vi "to string array.vi"(8 "error in (no error)":errorcluster, 11 "module configuration in":refnum<class "Daqmx Module configuration.lvclass">) -> (0 "error out":errorcluster, 1 "Array":string[][](array[string]), 2 "version":string, 3 "module configuration out":refnum<class "Daqmx Module configuration.lvclass">)   [LabVIEW 2015, in "DAQmx Module Configuration.lvclass"]
uses:
  Daqmx Module configuration.lvclass
  Daqmx Module configuration.lvclass/Daqmx Module configuration.ctl
  <vilib>/NI/Tag Bus/tag/tag descriptor.lvclass/tag descriptor.ctl
  <vilib>/NI/Tag Bus Module Framework/module configuration/TBM module configuration.lvclass
  <vilib>/NI/Tag Bus/tag/tag descriptor.lvclass
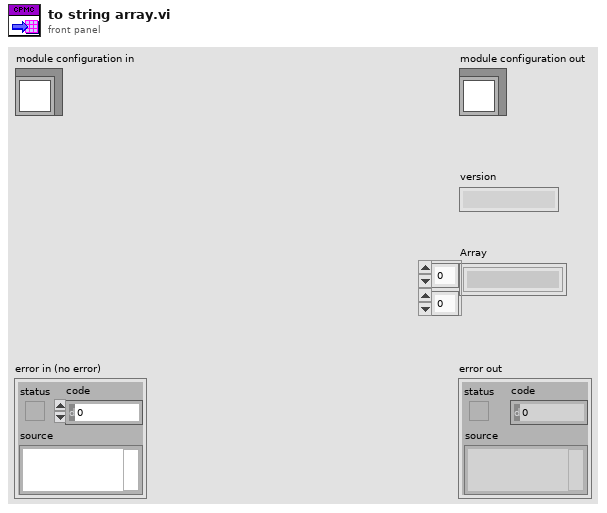
[diagram p1: front panel]
types:
  T1 = typedef "DAQmx Module Configuration.lvclass/Line.ctl" = cluster{"Channel Array":refnum<class "TBM channel.lvclass">[], "Physical Channel":string, "Measurement Type":T2, "Parameters":T3}
  T2 = typedef "DAQmx Module Configuration.lvclass/Measurement Type.ctl" = enum16{"Digital Input", "Digital Output", "Voltage Input", "Voltage Output", "Current Input", "Current Output", "RTD", "Thermocouple", "Strain", "PWM"}
  T3 = typedef "DAQmx Module Configuration.lvclass/Parameters.ctl" = cluster{"Digital Config":cluster{"Invert Lines?":bool}, "Voltage Config":cluster{"Maximum Value (V)":dbl, "Minimum Value (V)":dbl, "in terminal configuration (V)":i32, "out terminal configuration (V)":i32}, "Current Config":cluster{"Maximum Value (A)":dbl, "Minimum Value (A)":dbl, "shunt resistor location":i32, "input terminal configuration (C)":i32, "external shunt resistor value":dbl}, "RTD Config":cluster{"Maximum Value (°C)":dbl, "Minimum Value (°C)":dbl, "resistance configuration":i32, "r0":dbl, "current excitation value":dbl, "rtd type":i32, "current excitation source":i32}, "Thermocouple Config":cluster{"Minimum Value (C)":dbl, "Maximum Value (C)":dbl, "thermocouple type":i32, "cjc source":i32, "cjc value":dbl}, "Strain Config":cluster{"Maximum Value":dbl, "Minimum Value":dbl, "bridge information":cluster{"strain configuration":i32, "lead wire resistance":dbl, "initial bridge voltage":dbl, "voltage excitation source":i32, "voltage excitation value":dbl}, "strain gage information":cluster{"gage factor":dbl, "nominal gage resistance":dbl, "poisson ratio":dbl}}, "PWM Config":cluster{"Idle State":bool}}
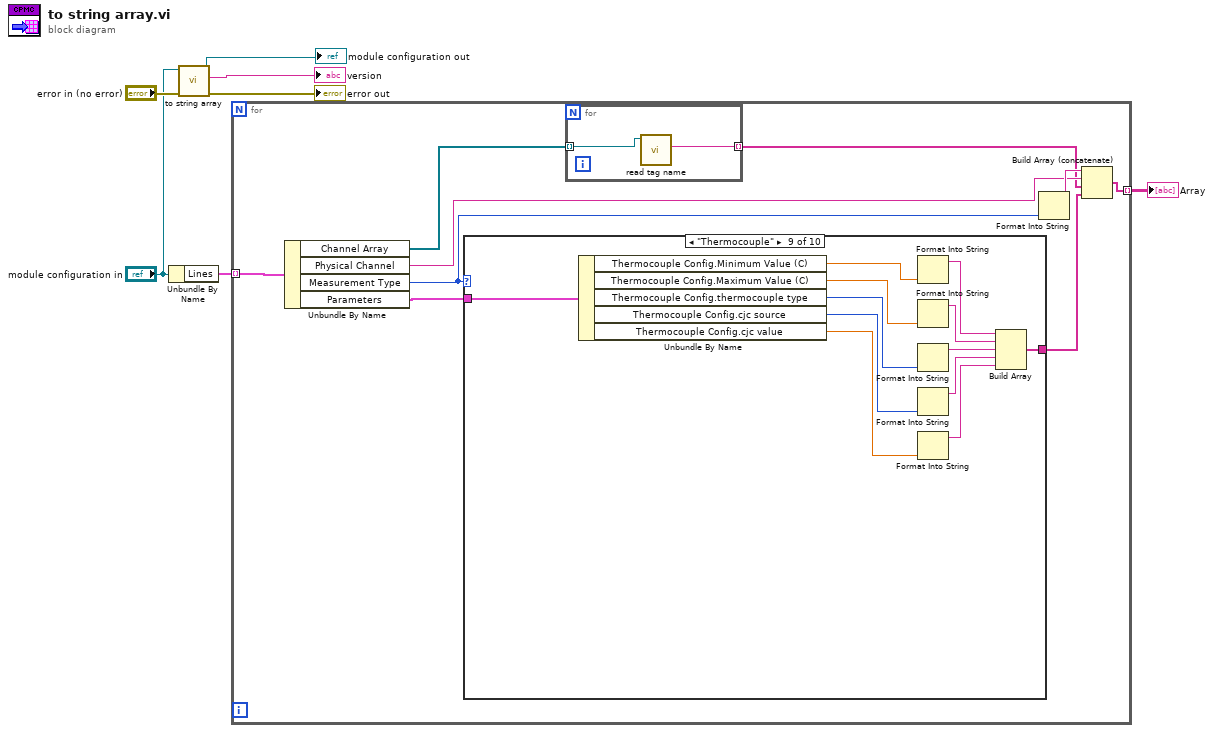
[diagram p0: block diagram]
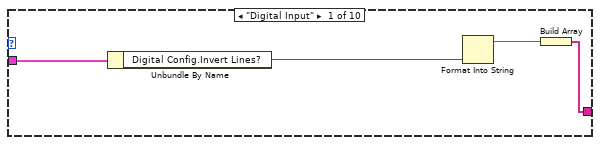
[diagram p2: hidden frame]
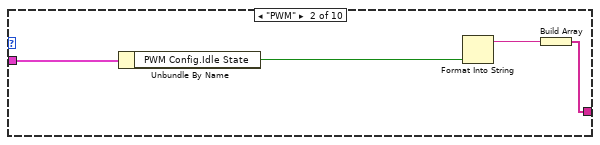
[diagram p3: hidden frame]
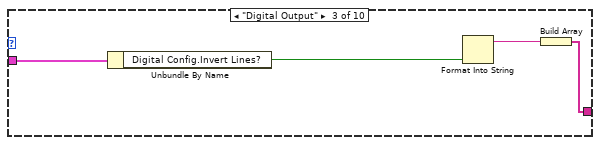
[diagram p4: hidden frame]
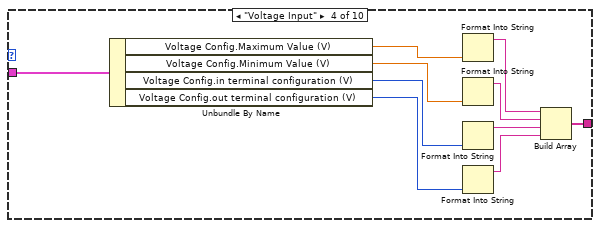
[diagram p5: hidden frame]
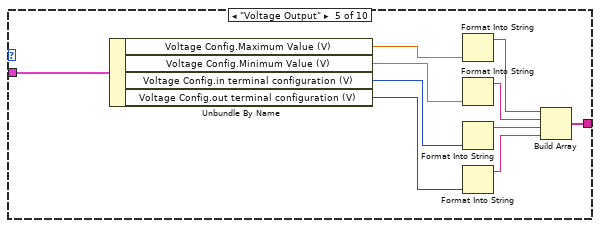
[diagram p6: hidden frame]
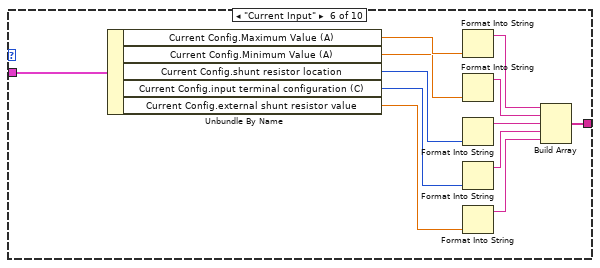
[diagram p7: hidden frame]
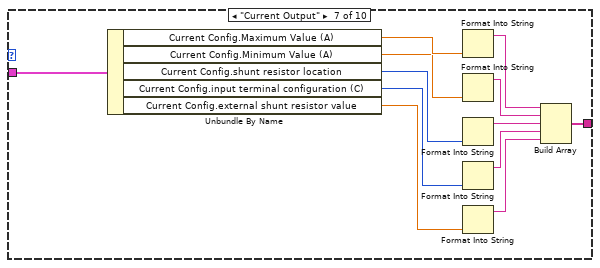
[diagram p8: hidden frame]
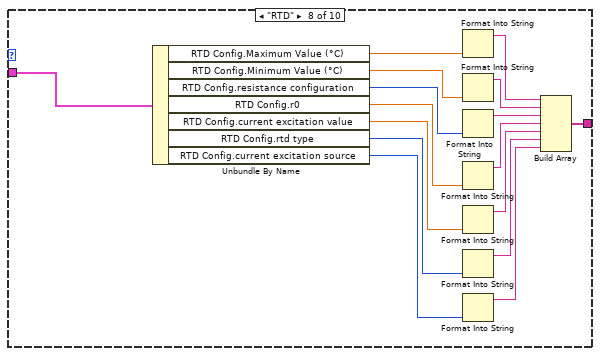
[diagram p9: hidden frame]
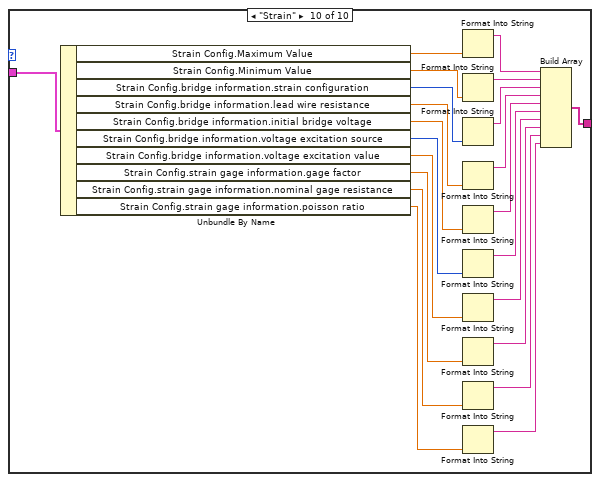
[diagram p10: hidden frame]
diagram:
  n1 = Unbundle By Name("module configuration in") -> ("Lines"=w2:T1[])
  n2 = call-parent "to string array.vi"("error in (no error)"="error in (no error)", "module configuration in"="module configuration in") -> ("error out"=→"error out":errorcluster, "version"=→"version":string, "module configuration out"=→"module configuration out":refnum<class "Daqmx Module configuration.lvclass">)  [unwired: 6 in, 1 out]
  n3 = for {
    tunnel: [w15] -> w1 mode=indexing
    tunnel: w2 -> [w16] mode=indexing
    n4 = Unbundle By Name(w16) -> ("Channel Array"=w11:refnum<class "TBM channel.lvclass">[], "Physical Channel"=w9:string, "Measurement Type"=w14:T2, "Parameters"=w13:T3)
    n5 = case shown="\"Thermocouple\"" w14 {
      tunnel: w13 -> [w22 w26 w30 w40 w50 w62 w74 w90 w102 w124]
      tunnel: [w19 w23 w27 w37 w47 w59 w71 w87 w99 w121] -> w12
      frame "Digital Input" {
        n6 = Unbundle By Name(w22) -> ("Digital Config.Invert Lines?"=w21:bool)
        n7 = Format Into String(w21) -> (resulting string=w20:string)  [unwired: 3 in, 1 out]
        n8 = Build Array(w20) -> (w19:string[])
      }
      frame "PWM" {
        n9 = Unbundle By Name(w26) -> ("PWM Config.Idle State"=w25:bool)
        n10 = Format Into String(w25) -> (resulting string=w24:string)  [unwired: 3 in, 1 out]
        n11 = Build Array(w24) -> (w23:string[])
      }
      frame "Digital Output" {
        n12 = Unbundle By Name(w30) -> ("Digital Config.Invert Lines?"=w29:bool)
        n13 = Format Into String(w29) -> (resulting string=w28:string)  [unwired: 3 in, 1 out]
        n14 = Build Array(w28) -> (w27:string[])
      }
      frame "Voltage Input" {
        n15 = Unbundle By Name(w40) -> ("Voltage Config.Maximum Value (V)"=w39:dbl, "Voltage Config.Minimum Value (V)"=w33:dbl, "Voltage Config.in terminal configuration (V)"=w32:i32, "Voltage Config.out terminal configuration (V)"=w31:i32)
        n16 = Format Into String(w39) -> (resulting string=w38:string)  [unwired: 3 in, 1 out]
        n17 = Format Into String(w33) -> (resulting string=w36:string)  [unwired: 3 in, 1 out]
        n18 = Format Into String(w32) -> (resulting string=w35:string)  [unwired: 3 in, 1 out]
        n19 = Format Into String(w31) -> (resulting string=w34:string)  [unwired: 3 in, 1 out]
        n20 = Build Array(w38, w36, w35, w34) -> (w37:string[])
      }
      frame "Voltage Output" {
        n21 = Unbundle By Name(w50) -> ("Voltage Config.Maximum Value (V)"=w49:dbl, "Voltage Config.Minimum Value (V)"=w43:dbl, "Voltage Config.in terminal configuration (V)"=w42:i32, "Voltage Config.out terminal configuration (V)"=w41:i32)
        n22 = Format Into String(w49) -> (resulting string=w48:string)  [unwired: 3 in, 1 out]
        n23 = Format Into String(w43) -> (resulting string=w46:string)  [unwired: 3 in, 1 out]
        n24 = Format Into String(w42) -> (resulting string=w45:string)  [unwired: 3 in, 1 out]
        n25 = Format Into String(w41) -> (resulting string=w44:string)  [unwired: 3 in, 1 out]
        n26 = Build Array(w48, w46, w45, w44) -> (w47:string[])
      }
      frame "Current Input" {
        n27 = Unbundle By Name(w62) -> ("Current Config.Maximum Value (A)"=w61:dbl, "Current Config.Minimum Value (A)"=w55:dbl, "Current Config.shunt resistor location"=w56:i32, "Current Config.input terminal configuration (C)"=w57:i32, "Current Config.external shunt resistor value"=w58:dbl)
        n28 = Format Into String(w61) -> (resulting string=w60:string)  [unwired: 3 in, 1 out]
        n29 = Format Into String(w55) -> (resulting string=w54:string)  [unwired: 3 in, 1 out]
        n30 = Format Into String(w56) -> (resulting string=w53:string)  [unwired: 3 in, 1 out]
        n31 = Format Into String(w57) -> (resulting string=w52:string)  [unwired: 3 in, 1 out]
        n32 = Format Into String(w58) -> (resulting string=w51:string)  [unwired: 3 in, 1 out]
        n33 = Build Array(w60, w54, w53, w52, w51) -> (w59:string[])
      }
      frame "Current Output" {
        n34 = Unbundle By Name(w74) -> ("Current Config.Maximum Value (A)"=w73:dbl, "Current Config.Minimum Value (A)"=w67:dbl, "Current Config.shunt resistor location"=w68:i32, "Current Config.input terminal configuration (C)"=w69:i32, "Current Config.external shunt resistor value"=w70:dbl)
        n35 = Format Into String(w73) -> (resulting string=w72:string)  [unwired: 3 in, 1 out]
        n36 = Format Into String(w67) -> (resulting string=w66:string)  [unwired: 3 in, 1 out]
        n37 = Format Into String(w68) -> (resulting string=w65:string)  [unwired: 3 in, 1 out]
        n38 = Format Into String(w69) -> (resulting string=w64:string)  [unwired: 3 in, 1 out]
        n39 = Format Into String(w70) -> (resulting string=w63:string)  [unwired: 3 in, 1 out]
        n40 = Build Array(w72, w66, w65, w64, w63) -> (w71:string[])
      }
      frame "RTD" {
        n41 = Unbundle By Name(w90) -> ("RTD Config.Maximum Value (°C)"=w89:dbl, "RTD Config.Minimum Value (°C)"=w86:dbl, "RTD Config.resistance configuration"=w77:i32, "RTD Config.r0"=w85:dbl, "RTD Config.current excitation value"=w84:dbl, "RTD Config.rtd type"=w83:i32, "RTD Config.current excitation source"=w82:i32)
        n42 = Format Into String(w89) -> (resulting string=w88:string)  [unwired: 3 in, 1 out]
        n43 = Format Into String(w86) -> (resulting string=w81:string)  [unwired: 3 in, 1 out]
        n44 = Format Into String(w77) -> (resulting string=w76:string)  [unwired: 3 in, 1 out]
        n45 = Format Into String(w85) -> (resulting string=w75:string)  [unwired: 3 in, 1 out]
        n46 = Format Into String(w84) -> (resulting string=w80:string)  [unwired: 3 in, 1 out]
        n47 = Format Into String(w83) -> (resulting string=w79:string)  [unwired: 3 in, 1 out]
        n48 = Format Into String(w82) -> (resulting string=w78:string)  [unwired: 3 in, 1 out]
        n49 = Build Array(w88, w81, w76, w75, w80, w79, w78) -> (w87:string[])
      }
      frame "Thermocouple" {
        n50 = Unbundle By Name(w102) -> ("Thermocouple Config.Minimum Value (C)"=w101:dbl, "Thermocouple Config.Maximum Value (C)"=w98:dbl, "Thermocouple Config.thermocouple type"=w97:i32, "Thermocouple Config.cjc source"=w96:i32, "Thermocouple Config.cjc value"=w95:dbl)
        n51 = Format Into String(w101) -> (resulting string=w100:string)  [unwired: 3 in, 1 out]
        n52 = Format Into String(w98) -> (resulting string=w94:string)  [unwired: 3 in, 1 out]
        n53 = Format Into String(w97) -> (resulting string=w93:string)  [unwired: 3 in, 1 out]
        n54 = Format Into String(w96) -> (resulting string=w92:string)  [unwired: 3 in, 1 out]
        n55 = Format Into String(w95) -> (resulting string=w91:string)  [unwired: 3 in, 1 out]
        n56 = Build Array(w100, w94, w93, w92, w91) -> (w99:string[])
      }
      frame "Strain" {
        n57 = Unbundle By Name(w124) -> ("Strain Config.Maximum Value"=w123:dbl, "Strain Config.Minimum Value"=w120:dbl, "Strain Config.bridge information.strain configuration"=w119:i32, "Strain Config.bridge information.lead wire resistance"=w118:dbl, "Strain Config.bridge information.initial bridge voltage"=w117:dbl, "Strain Config.bridge information.voltage excitation source"=w116:i32, "Strain Config.bridge information.voltage excitation value"=w110:dbl, "Strain Config.strain gage information.gage factor"=w109:dbl, "Strain Config.strain gage information.nominal gage resistance"=w108:dbl, "Strain Config.strain gage information.poisson ratio"=w107:dbl)
        n58 = Format Into String(w123) -> (resulting string=w122:string)  [unwired: 3 in, 1 out]
        n59 = Format Into String(w120) -> (resulting string=w115:string)  [unwired: 3 in, 1 out]
        n60 = Format Into String(w119) -> (resulting string=w114:string)  [unwired: 3 in, 1 out]
        n61 = Format Into String(w118) -> (resulting string=w113:string)  [unwired: 3 in, 1 out]
        n62 = Format Into String(w117) -> (resulting string=w112:string)  [unwired: 3 in, 1 out]
        n63 = Format Into String(w116) -> (resulting string=w111:string)  [unwired: 3 in, 1 out]
        n64 = Format Into String(w110) -> (resulting string=w106:string)  [unwired: 3 in, 1 out]
        n65 = Format Into String(w109) -> (resulting string=w105:string)  [unwired: 3 in, 1 out]
        n66 = Format Into String(w108) -> (resulting string=w104:string)  [unwired: 3 in, 1 out]
        n67 = Format Into String(w107) -> (resulting string=w103:string)  [unwired: 3 in, 1 out]
        n68 = Build Array(w122, w115, w114, w113, w112, w111, w106, w105, w104, w103) -> (w121:string[])
      }
    }
    n69 = for {
      tunnel: [w18] -> w8 mode=indexing
      tunnel: w11 -> [w17] mode=indexing
      n70 = call <vilib>:"read tag name.vi"("system tag in"=w17) -> ("name"=w18:string)  [unwired: 8 in, 2 out]
    }
    n71 = Format Into String(w14) -> (resulting string=w10:string)  [unwired: 3 in, 1 out]
    n72 = Build Array (concatenate)(w10, w9, w8, w12) -> (w15:string[])
  }
  "Array" <- w1
